vi "FromRepo.vi"(8 "error in":errorcluster, 9 "from repo cluster":T2, 10 "repository in":refnum<class "NISE_CEF_Repository.lvclass">, 11 "node in":refnum<class "NISE_CEF_Node.lvclass">) -> (0 "error out":errorcluster, 2 "repository out":refnum<class "NISE_CEF_Repository.lvclass">, 3 "node":T1)   [LabVIEW 2014, in "NISE_CEF_Node.lvclass"]
doc: "Grabs information from the Repo and stores it in the nodes."
uses:
  NISE_CEF_Node.lvclass
  Repository/NISE_CEF_Repository.lvclass
  FromRepoCluster.ctl
  NodeRef.ctl
  NISE_CEF_Node.lvclass/NISE_CEF_Node.ctl
  WriteParent.vi
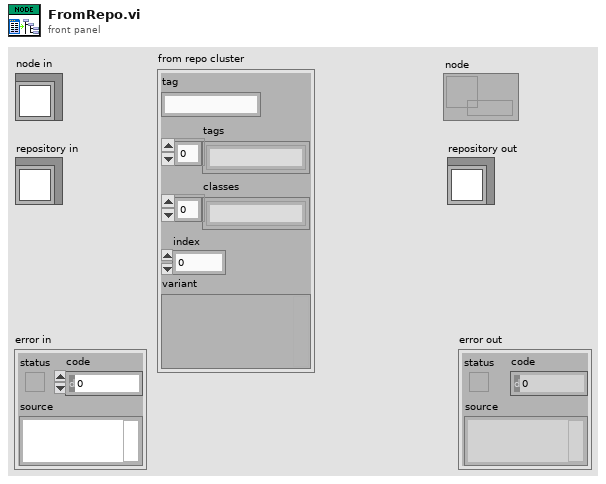
[diagram p1: front panel]
types:
  T1 = typedef "NISE_CEF_Node.lvclass/NodeRef.ctl" = refnum<data-value>
  T2 = typedef "NISE_CEF_Node.lvclass/FromRepoCluster.ctl" = cluster{"tag":string, "tags":string[], "classes":string[], "index":i32, "variant":variant}
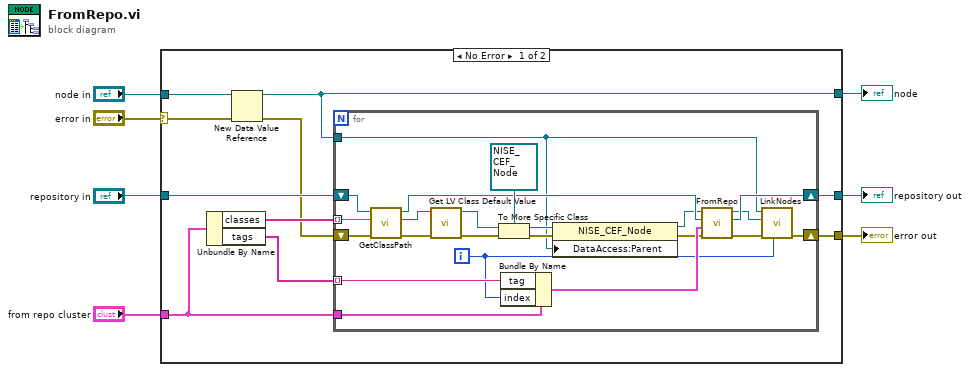
[diagram p0: block diagram]
diagram:
  n1 = case shown="No Error" "error in" {
    selector: "error in" -> [w9 w41]
    tunnel: [w16 w41] -> w6
    tunnel: "node in" -> [w14 _]
    tunnel: "repository in" -> [w10 w40]
    tunnel: [w15 w40] -> w3
    tunnel: "from repo cluster" -> [w11 _]
    tunnel: [w13 _] -> w1
    frame No Error {
      n2 = Unbundle By Name(w11) -> ("classes"=w17:string[], "tags"=w12:string[])
      n3 = New Data Value Reference(data value=w14, error in=w9) -> (data value reference=w13:refnum<data-value>, error out=w8:errorcluster)
      n4 = for {
        tunnel: w17 -> [w22] mode=indexing
        shift-right: [w35] -> w15
        shift-left: w10 -> [w27]
        shift-right: [w32] -> w16
        shift-left: w8 -> [w26]
        tunnel: w13 -> [w18]
        tunnel: w12 -> [w30] mode=indexing
        tunnel: w11 -> [w29]
        i -> [w28]
        n5 = call-dynamic "GetClassPath.vi"("error in"=w26, "class name"=w22, "Repository in"=w27) -> ("error out"=w25:errorcluster, "class path"=w24:path, "Repository out"=w23:refnum<class "NISE_CEF_Repository.lvclass">)  [unwired: 6 in]
        n6 = call <vilib>:"Get LV Class Default Value.vi"("error in (no error)"=w25, "class path"=w24) -> ("error out"=w37:errorcluster, "object"=w38:refnum<class>)  [unwired: 8 in]
        n7 = To More Specific Class(target class=refnum<class "NISE_CEF_Node.lvclass"> refnum ("node.lvclass"), reference=w38, error in=w37) -> (specific class reference=w20:refnum<class "NISE_CEF_Node.lvclass">, error out=w36:errorcluster)
        n8 = Bundle By Name(cluster=w29, "tag"=w30, "index"=w28) -> (w31:T2)
        n9 = property class="NISE_CEF_Node"(reference=w20, error in=w36, "DataAccess:Parent"=w18) -> (reference out=w19:refnum<class "NISE_CEF_Node.lvclass">, error out=w21:errorcluster)
        n10 = call-dynamic "FromRepo.vi"("error in"=w21, "from repo cluster"=w31, "repository in"=w23, "node in"=w19) -> ("error out"=w33:errorcluster, "repository out"=w35:refnum<class "NISE_CEF_Repository.lvclass">, "node"=w34:T1)  [unwired: 5 in]
        n11 = call "LinkNodes.vi"("index"=w28, "error in"=w33, "child in"=w34, "parent in"=w18) -> ("error out"=w32:errorcluster)  [unwired: 5 in, 2 out]
      }
    }
    frame Error {
    }
  }
  "error out" <- w6
  "repository out" <- w3
  "node" <- w1
